vi "clone.vi"(0 "reference":refnum<class "StateNode.lvclass">, 5 "error in (no error)":errorcluster) -> (14 "reference out":refnum<class "StateNode.lvclass">, 15 "clonedInterfaceNode":refnum<class "AbstractNode.lvclass">, 19 "error out":errorcluster)   [LabVIEW 2020, in "StateNode.lvclass"]
doc: "public Object clone()"
uses:
  <resource>/Framework/Providers/Open_GDS/UML/StateNode_class/StateNode.lvclass
  C:/Program Files (x86)/National Instruments/LabVIEW 2020/resource/Framework/Providers/Open_GDS/UML/RectangularNode_class/RectangularNode.lvclass
  C:/Program Files (x86)/National Instruments/LabVIEW 2020/resource/Framework/Providers/Open_GDS/UML/AbstractNode_class/AbstractNode.lvclass
  <resource>/Framework/Providers/Open_GDS/UML/AbstractNode_class/AbstractNode.lvclass
  <resource>/Framework/Providers/Open_GDS/UML/MultiLineString_class/MultiLineString.lvclass
  <resource>/Framework/Providers/Open_GDS/UML/RectangularNode_class/RectangularNode.lvclass
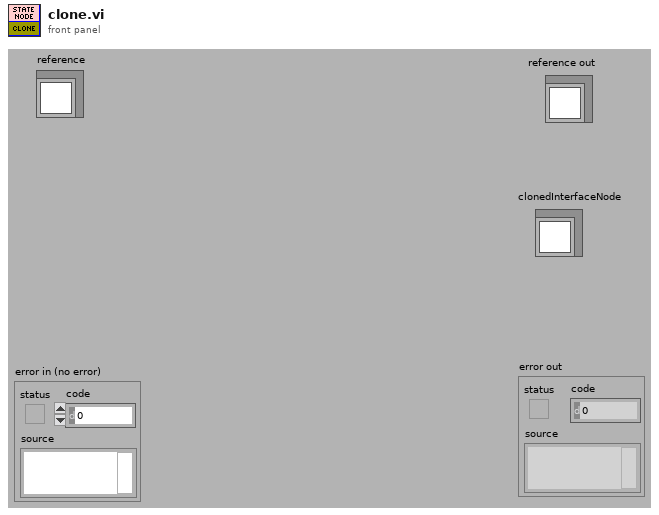
[diagram p1: front panel]
types:
  T1 = typedef "RectangularNode.lvclass/ObjectAttributes.ctl" = cluster{"bounds":T2}
  T2 = typedef "Rectangle Rectangle2D.ctl" = cluster{"x":dbl, "y":dbl, "width":dbl, "height":dbl}
  T3 = typedef "StateNode.lvclass/ObjectAttributes.ctl" = cluster{"state":refnum<class "MultiLineString.lvclass">, "action":refnum<class "MultiLineString.lvclass">, "DEFAULT_WIDTH":i32, "DEFAULT_HEIGHT":i32}
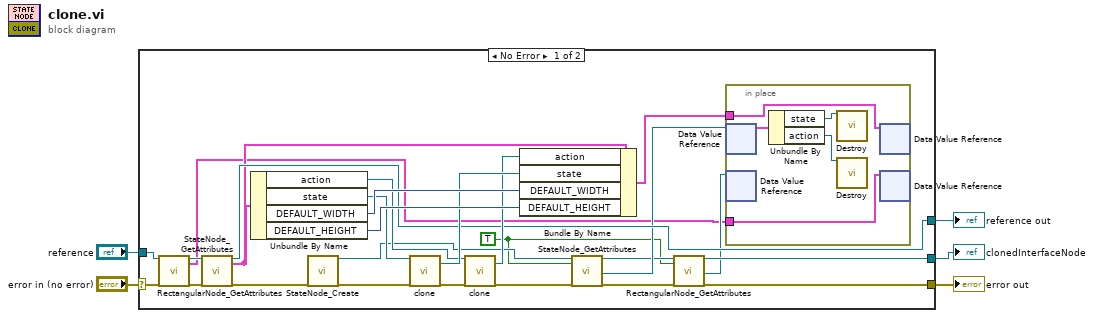
[diagram p0: block diagram]
diagram:
  n1 = case shown="No Error" "error in (no error)" {
    selector: "error in (no error)" -> [w31 w37]
    tunnel: "reference" -> [w13 w38]
    tunnel: [w11 w37] -> w4
    tunnel: [w20 w38] -> w3
    tunnel: [w9 _] -> w1
    frame No Error {
      w6 = TRUE ("OnlyGetDvrReference(False)")
      n2 = call <resource>:"RectangularNode_GetAttributes.vi"("reference in"=w13, "error in (no error)"=w31) -> ("reference out"=w12:refnum<class "StateNode.lvclass">, "Data"=w7:T1, "error out"=w14:errorcluster)  [unwired: 14 in, 1 out]
      n3 = call <resource>:"StateNode_GetAttributes.vi"("reference in"=w12, "error in (no error)"=w14) -> ("reference out"=w20:refnum<class "StateNode.lvclass">, "Data"=w18:T3, "error out"=w19:errorcluster)  [unwired: 1 in, 14 out]
      n4 = Unbundle By Name(w18) -> ("action"=w24:refnum<class "MultiLineString.lvclass">, "state"=w27:refnum<class "MultiLineString.lvclass">, "DEFAULT_WIDTH"=w30:i32, "DEFAULT_HEIGHT"=w29:i32)
      n5 = call <resource>:"StateNode_Create.vi"("error in (no error)"=w19) -> ("reference out"=w21:refnum<class "StateNode.lvclass">, "error out"=w28:errorcluster)  [unwired: 17 in]
      n6 = call-dynamic "clone.vi"("reference"=w27, "error in (no error)"=w28) -> ("clonedMultiLineString"=w26:refnum<class "MultiLineString.lvclass">, "error out"=w25:errorcluster)  [unwired: 15 in, 1 out]
      n7 = call-dynamic "clone.vi"("reference"=w24, "error in (no error)"=w25) -> ("clonedMultiLineString"=w23:refnum<class "MultiLineString.lvclass">, "error out"=w22:errorcluster)  [unwired: 15 in, 1 out]
      n8 = Bundle By Name(cluster=w18, "action"=w23, "state"=w26, "DEFAULT_WIDTH"=w30, "DEFAULT_HEIGHT"=w29) -> (w16:T3)
      n9 = call <resource>:"StateNode_GetAttributes.vi"("reference in"=w21, "OnlyGetDvrReference(False)"=w6, "error in (no error)"=w22) -> ("reference out"=w10:refnum<class "StateNode.lvclass">, "DataRef"=w17:refnum<data-value>, "error out"=w15:errorcluster)  [unwired: 13 in, 1 out]
      n10 = call <resource>:"RectangularNode_GetAttributes.vi"("reference in"=w10, "OnlyGetDvrReference(False)"=w6, "error in (no error)"=w15) -> ("reference out"=w9:refnum<class "StateNode.lvclass">, "DataRef"=w8:refnum<data-value>, "error out"=w11:errorcluster)  [unwired: 13 in, 1 out]
      n11 = in-place {
        in-place-border: w16 -> [w36]
        in-place-border: w7 -> [w32]
        n12 = in-place-dvr #1(w17) -> (w34:T3)  [unwired: 1 out]
        n13 = in-place-dvr #2(w8) -> ()  [unwired: 2 out]
        n14 = Unbundle By Name(w34) -> ("state"=w35:refnum<class "MultiLineString.lvclass">, "action"=w33:refnum<class "MultiLineString.lvclass">)
        n15 = call-dynamic "Destroy.vi"("reference"=w35) -> ()  [unwired: 17 in, 2 out]
        n16 = call-dynamic "Destroy.vi"("reference"=w33) -> ()  [unwired: 17 in, 2 out]
        n17 = in-place-dvr #1(w36) -> ()  [unwired: 2 out]
        n18 = in-place-dvr #2(w32) -> ()  [unwired: 2 out]
      }
    }
    frame Error {
    }
  }
  "reference out" <- w3
  "error out" <- w4
  "clonedInterfaceNode" <- w1
